vi "Demo.vi"(6 "1D Array double In":dbl[](array[numeric])=[1.1, 2.2, 3.3], 7 "Offset":dbl=-5.0, 9 "ComplexDouble In":cdb=11.22+33.44i, 10 "Double In":dbl=111.111, 11 "Int32 In":i32=123) -> (1 "ComplexDouble Out":cdb=246.0+0.0i, 2 "Double Out":dbl, 3 "Int32 Out":i32=246, 4 "1D Array double Out":dbl[](array[numeric]))   [LabVIEW 2012]
panel:
  # "Int32 Out = Int32 In + Offset"
  # "Double Out = Double In + Offset"
  # "ComplexDouble Out = ComplexDouble In + Offset"
  # "1D Array double Out = - 1D Array double In"
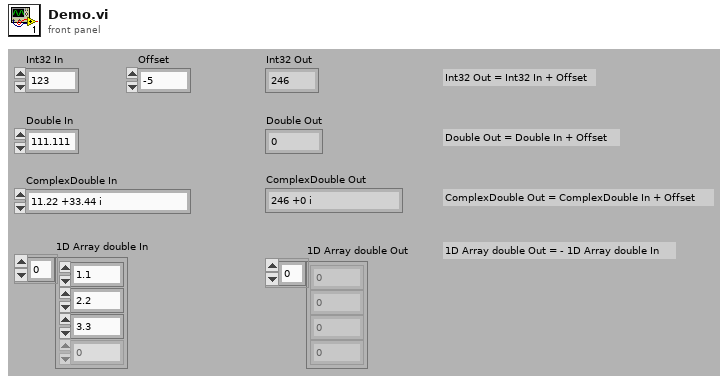
[diagram p1: front panel]
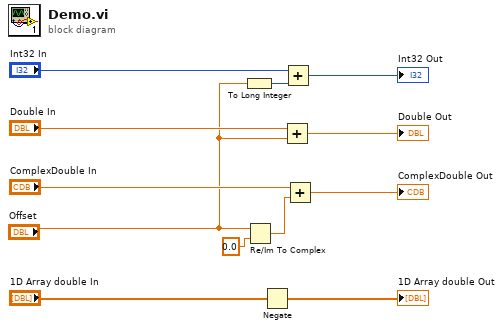
[diagram p0: block diagram]
diagram:
  n1 = To Long Integer(number="Offset") -> (32bit integer=w4:i32)
  n2 = Re/Im To Complex(1:0.0 ("y"), 2:"Offset") -> (0:w2:cdb)
  n3 = Negate(x="1D Array double In") -> (-x=→"1D Array double Out":dbl[])
  n4 = Add(x="Double In", y="Offset") -> (x+y=→"Double Out":dbl)
  n5 = Add(x="Int32 In", y=w4) -> (x+y=→"Int32 Out":i32)
  n6 = Add(x="ComplexDouble In", y=w2) -> (x+y=→"ComplexDouble Out":cdb)
